vi "Event Handler.vi"(0 "uService Template in":refnum<class "Error Manager.lvclass">, 5 "Event type":T1=enum."Message", 7 "Item Name":string, 9 "Data":variant, 11 "error in (no error)":errorcluster) -> (4 "uService Template out":refnum<class "Error Manager.lvclass">, 15 "error out":errorcluster)   [LabVIEW 2020, in "TALOS.lvlib" / "Error Manager.lvlib" / "Error Manager.lvclass"]
doc: "This VI is the event handler of the uService: every time an event is triggered to the uService, this VI is called.\nNote: here you can access the Actor/Class data, but it will be the one coming out from Init. You cannot modify the values.\nThree different events are supported:\nI) Button Pressed: get called on a GUI button pressed. Item Name is the name (label) of the button, Data is empty.\nII) Shared Variable Updated: get called when a SV you subscribed to is updated. Item Name is the name of the SV, and Data is the value (note: you need to convert it to the proper type).\nIII) Message: get called every time a user event is generated using Send Message to Event Handler. The values of Item Name and Data are the one given to the Send Message to Event Handler.\nIV) Ready to launch?: this frame get called every time a new Run is initiated. Each uService is responsible of performing a self check before giving back the green light for the Run to start."
uses:
  Error Manager.lvclass
  C:/Users/marco/Documents/GitHub_Lab/TALOS/talos/Father of all uServices/Father of all uServices/Father of all uServices.lvclass
  Father of all uServices/Father of all uServices/Event Handler Items.ctl
  Ancestor/Ancestor/Ancestor.lvclass/Ancestor.ctl
  Error Manager Consumer Case Selector.ctl
  Father of all uServices/Father of all uServices Messages/Consumer Msg/Consumer Msg.lvclass/Consumer Msg.ctl
  Error Info.ctl
  Father of all uServices/Father of all uServices/Father of all uServices.lvclass/Father of all uServices.ctl
  FGV/Error Memory/Get Error Description.vi
  Support VIs/Get PC name.vi
  Ancestor/Ancestor/Read ID.vi
  Support VIs/Get Class Name.vi
  <vilib>/Utility/error.llb/Clear Errors.vi
  Father of all uServices/Father of all uServices Messages/Consumer Msg/Send Consumer.vi
  FGV/Error Memory/Error Memory Core.vi
  <vilib>/AdvancedString/Delimited String to 1D String Array.vi
  Support VIs/Circus Root Path.vi
  FGV/Error Memory/Error Crt Lvl checker.vi
  FGV/Error Memory/Error Memory Core.vi/40c8088d-b597-4017-91af-faa98e00292e.vi
  FGV/Error Memory/Error Memory Core.vi/d4a3ab98-063c-4e44-b43d-fbdcfe6c2be2.vi
  Father of all uServices/Father of all uServices/Father of all uServices.lvclass
  C:/Users/marco/Documents/GitHub_Lab/TALOS/builds/Actor Framework PPL/Actor Framework.lvlibp/1abvi3w/vi.lib/ActorFramework/Actor/Actor.lvclass
  Support VIs/Global Memory.vi
  <vilib>/Utility/LVClass/Get LV Class Name.vi
  Support VIs/Is in Packed Library.vi
  Support VIs/TALOS Root path.vi
  Support VIs/Read CSV worksheet.vi
  Support VIs/Global Constants.vi
  <vilib>/Utility/error.llb/General Error Handler.vi
  Support VIs/Error Log.vi
  builds/Actor Framework PPL/Actor Framework.lvlibp/1abvi3w/vi.lib/ActorFramework/Actor/Read Self Enqueuer.vi
  <userlib>/_OpenG.lib/lvdata/lvdata.llb/Get Strings from Enum__ogtk.vi
  builds/Actor Framework PPL/Actor Framework.lvlibp/1abvi3w/vi.lib/ActorFramework/Message Enqueuer/Enqueue.vi
  Ancestor/Ancestor/Ancestor.lvclass
  <vilib>/Comparison/Equal/Equal Functor/Equal Functor.lvclass
  Father of all uServices/Father of all uServices Messages/Consumer Msg/Consumer Msg.lvclass
  Error Manager.lvclass/Error Manager.ctl
  TALOS.lvlib
  FGV/Error Memory/Error Memory.lvlib
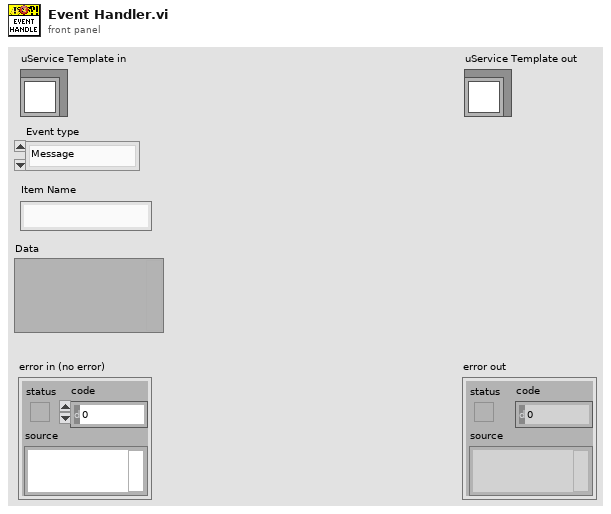
[diagram p1: front panel]
types:
  T1 = typedef "TALOS.lvlib/Father of all uServices.lvlib/Father of all uServices.lvclass/Event Handler Items.ctl" = enum16{"Button Pressed", "Message", "Ready to launch?", "Safe Mode", "Start RUN", "Stop RUN"}
  T2 = typedef "TALOS.lvlib/Error Manager.lvlib/Error Manager.lvclass/Error Manager Consumer Case Selector.ctl" = enum16{"Init", "Digest Error", "Dismiss Error", "Dismiss All", "Show Error Details", "Filter out Errors", "Clear Filters"}
  T3 = typedef "TALOS.lvlib/Error Manager.lvlib/Error Manager.lvclass/Error Info.ctl" = cluster{"error out":errorcluster, "Time Stamp":timestamp, "Machine Name":string, "GUID":string}
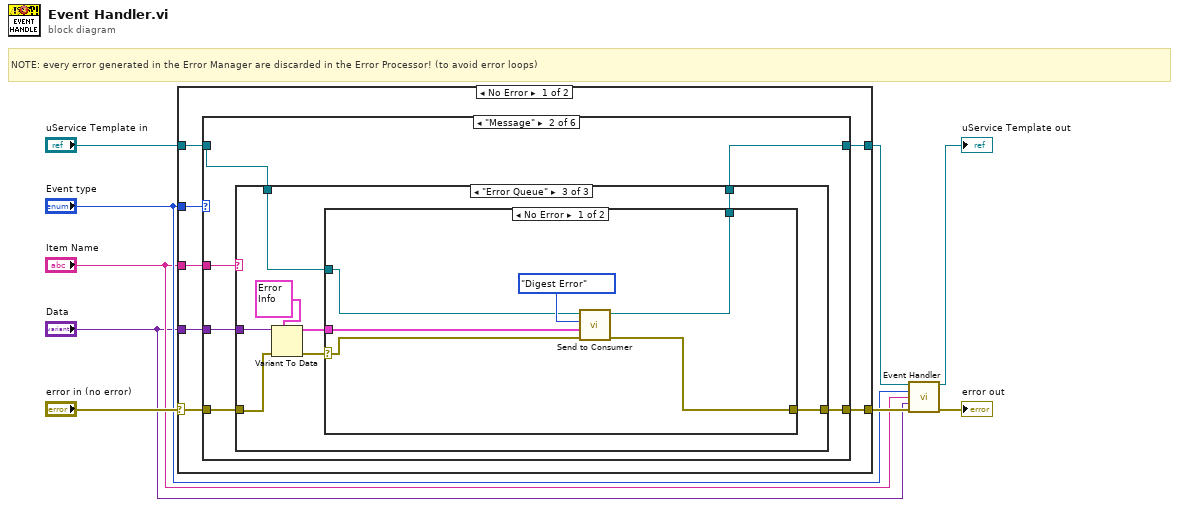
[diagram p0: block diagram]
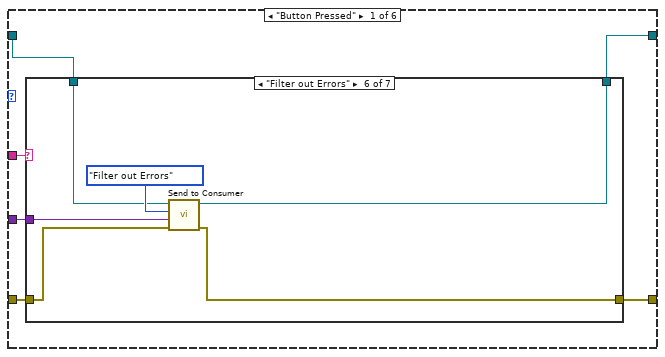
[diagram p2: hidden frame]
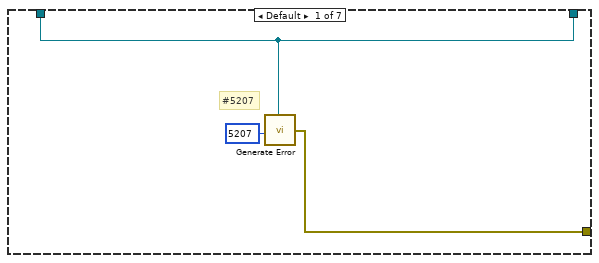
[diagram p3: hidden frame]
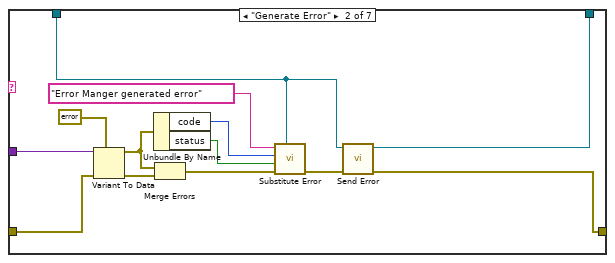
[diagram p4: hidden frame]
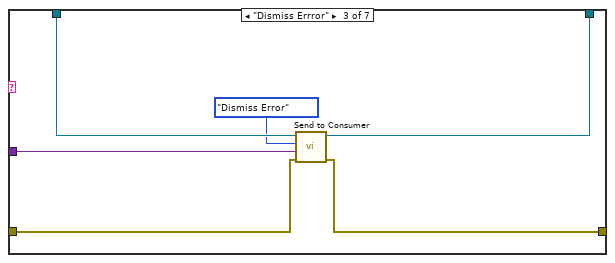
[diagram p5: hidden frame]
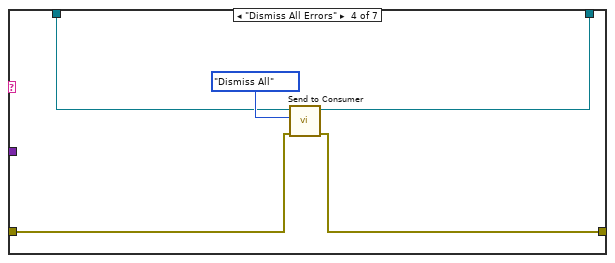
[diagram p6: hidden frame]
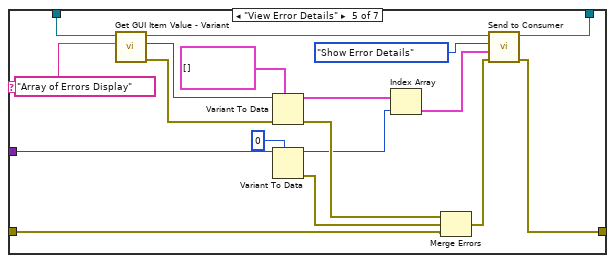
[diagram p7: hidden frame]
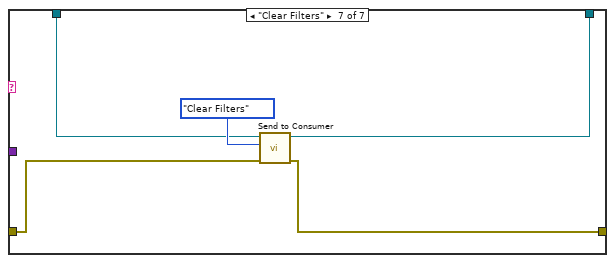
[diagram p8: hidden frame]
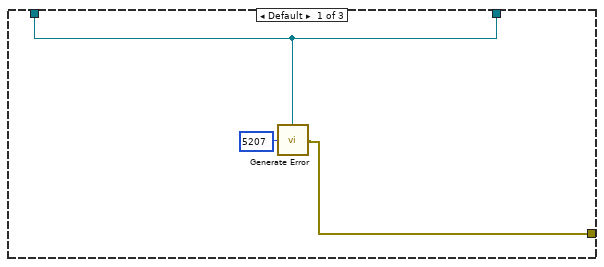
[diagram p9: hidden frame]
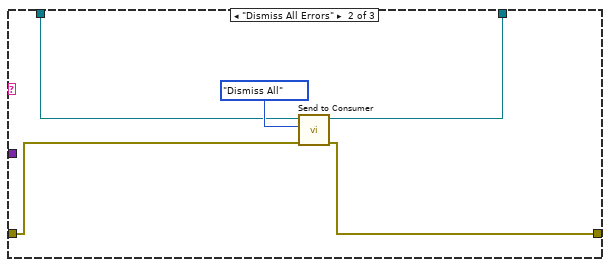
[diagram p10: hidden frame]
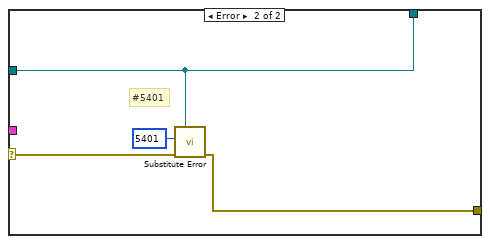
[diagram p11: hidden frame]
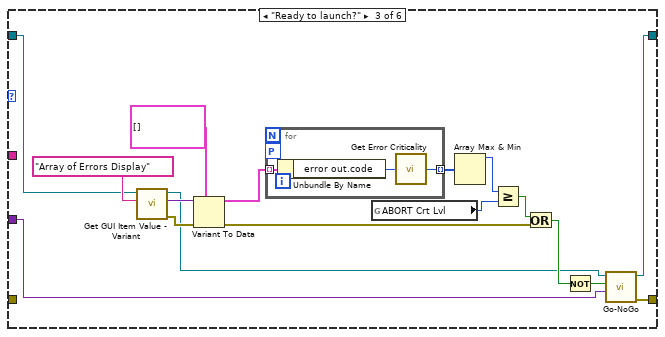
[diagram p12: hidden frame]
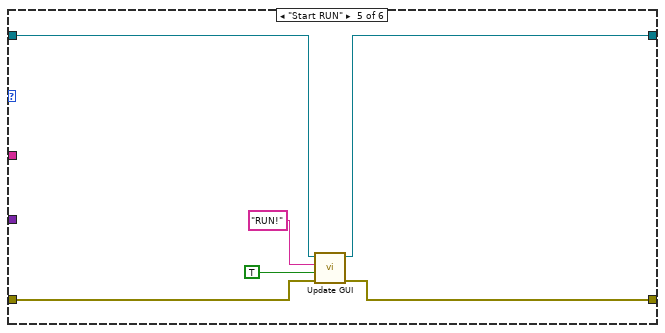
[diagram p14: hidden frame]
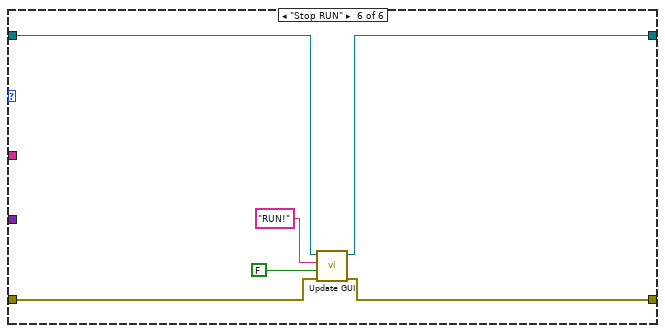
[diagram p15: hidden frame]
diagram:
  # "NOTE: every error generated in the Error Manager are discarded in the Error Processor! (to avoid error loops)"
  n1 = case shown="No Error" "error in (no error)" {
    selector: "error in (no error)" -> [w14 w146]
    tunnel: [w15 w146] -> w7
    tunnel: [w10 w145] -> w4
    tunnel: "uService Template in" -> [w13 w145]
    tunnel: "Event type" -> [w16 _]
    tunnel: "Item Name" -> [w12 _]
    tunnel: "Data" -> [w11 _]
    frame No Error {
      n2 = case shown="\"Message\"" w16 {
        tunnel: [w22 w80 w124 w132 w138 w144] -> w15
        tunnel: w14 -> [w19 w84 _ w132 w137 w143]
        tunnel: w12 -> [w20 w83 _ _ _ _]
        tunnel: w13 -> [w21 w81 w123 w131 w134 w140]
        tunnel: w11 -> [w18 w82 w113 _ _ _]
        tunnel: [w17 w79 w111 w131 w133 w139] -> w10
        frame "Button Pressed" {
          n3 = case shown="\"Filter out Errors\"" w20 {
            tunnel: w19 -> [_ w36 w42 w47 w52 w71 w76]
            tunnel: [w24 w37 w41 w46 w59 w70 w75] -> w22
            tunnel: w21 -> [w23 w33 w44 w48 w63 w72 w77]
            tunnel: w18 -> [_ w34 w40 _ w57 w69 _]
            tunnel: [w23 w26 w39 w45 w50 w68 w74] -> w17
            frame Default {
              # "#5207"
              n4 = call "Generate Error.vi"("Class"=w23, "Error Code"=5207) -> ("error out"=w24:errorcluster)  [unwired: 5 in]
            }
            frame "Generate Error" {
              n5 = Variant To Data(error in=w36, type=errorcluster {"status"=FALSE, "code"=0, "source"=""} ("error IO"), Variant=w34) -> (data=w30:errorcluster, error out=w38:errorcluster)
              n6 = Unbundle By Name(w30) -> ("code"=w29:i32, "status"=w28:bool)
              n7 = Merge Errors(w30, w38) -> (w32:errorcluster)
              n8 = call "Substitute Error.vi"("LabVIEW Object"=w33, "error in (no error)"=w32, "Error/Warning"=w28, "Error Code"=w29, "Optional String"="Error Manger generated error") -> ("error out"=w31:errorcluster)  [unwired: 6 in]
              n9 = call-dynamic "Send Error.vi"("error in (no error)"=w31, "Father of all uServices in"=w33) -> ("error out"=w37:errorcluster, "Father of all uServices out"=w26:refnum<class "Error Manager.lvclass">)  [unwired: 8 in]
            }
            frame "Dismiss Errror" {
              n10 = call "Send to Consumer.vi"("error in (no error)"=w42, "Data"=w40, "Case ID"=Error_Manager_Consumer_Case_Selector."Dismiss Error" ("ErrMgr Case Selector"), "uService Template in"=w44) -> ("error out"=w41:errorcluster, "uService Template out"=w39:refnum<class "Error Manager.lvclass">)  [unwired: 6 in]
            }
            frame "Dismiss All Errors" {
              n11 = call "Send to Consumer.vi"("error in (no error)"=w47, "Case ID"=Error_Manager_Consumer_Case_Selector."Dismiss All" ("ErrMgr Case Selector"), "uService Template in"=w48) -> ("error out"=w46:errorcluster, "uService Template out"=w45:refnum<class "Error Manager.lvclass">)  [unwired: 7 in]
            }
            frame "View Error Details" {
              n12 = call "Get GUI Item Value - Variant.vi"("FP Item Name"="Array of Errors Display", "uService Template in"=w63) -> ("error out"=w62:errorcluster, "Value"=w61:variant, "uService Template out"=w58:refnum<class "Error Manager.lvclass">)  [unwired: 7 in]
              n13 = Variant To Data(error in=w62, type=T3[] [] ("error constant"), Variant=w61) -> (data=w65:T3[], error out=w67:errorcluster)
              n14 = Variant To Data(type=0 ("Select Error"), Variant=w57) -> (data=w54:i32, error out=w53:errorcluster)  [unwired: 1 in]
              n15 = Index Array(array=w65, index=w54) -> (element=w55:T3)
              n16 = Merge Errors(w67, w53, w52) -> (w51:errorcluster)
              n17 = call "Send to Consumer.vi"("error in (no error)"=w51, "Data"=w55, "Case ID"=Error_Manager_Consumer_Case_Selector."Show Error Details" ("ErrMgr Case Selector"), "uService Template in"=w58) -> ("error out"=w59:errorcluster, "uService Template out"=w50:refnum<class "Error Manager.lvclass">)  [unwired: 6 in]
            }
            frame "Filter out Errors" {
              n18 = call "Send to Consumer.vi"("error in (no error)"=w71, "Data"=w69, "Case ID"=Error_Manager_Consumer_Case_Selector."Filter out Errors" ("ErrMgr Case Selector"), "uService Template in"=w72) -> ("error out"=w70:errorcluster, "uService Template out"=w68:refnum<class "Error Manager.lvclass">)  [unwired: 6 in]
            }
            frame "Clear Filters" {
              n19 = call "Send to Consumer.vi"("error in (no error)"=w76, "Case ID"=Error_Manager_Consumer_Case_Selector."Clear Filters" ("ErrMgr Case Selector"), "uService Template in"=w77) -> ("error out"=w75:errorcluster, "uService Template out"=w74:refnum<class "Error Manager.lvclass">)  [unwired: 7 in]
            }
          }
        }
        frame "Message" {
          n20 = case shown="\"Error Queue\"" w83 {
            tunnel: w84 -> [_ w90 w95]
            tunnel: w82 -> [_ _ w94]
            tunnel: w81 -> [w85 w91 w96]
            tunnel: [w87 w89 w97] -> w80
            tunnel: [w85 w88 w93] -> w79
            frame Default {
              n21 = call "Generate Error.vi"("Class"=w85, "Error Code"=5207) -> ("error out"=w87:errorcluster)  [unwired: 5 in]
            }
            frame "Dismiss All Errors" {
              n22 = call "Send to Consumer.vi"("error in (no error)"=w90, "Case ID"=Error_Manager_Consumer_Case_Selector."Dismiss All" ("ErrMgr Case Selector"), "uService Template in"=w91) -> ("error out"=w89:errorcluster, "uService Template out"=w88:refnum<class "Error Manager.lvclass">)  [unwired: 7 in]
            }
            frame "Error Queue" {
              n23 = Variant To Data(error in=w95, type=T3 {"error out"={"status"=FALSE, "code"=0, "source"=""}, "Time Stamp"=timestamp(0 s since 1904-01-01), "Machine Name"="", "GUID"=""} ("Error Info"), Variant=w94) -> (data=w99:T3, error out=w100:errorcluster)
              n24 = case shown="No Error" w100 {
                selector: w100 -> [w105 w110]
                tunnel: w96 -> [w102 w107]
                tunnel: [w106 w109] -> w97
                tunnel: w99 -> [w104 _]
                tunnel: [w101 w107] -> w93
                frame No Error {
                  n25 = call "Send to Consumer.vi"("error in (no error)"=w105, "Data"=w104, "Case ID"=Error_Manager_Consumer_Case_Selector."Digest Error" ("ErrMgr Case Selector"), "uService Template in"=w102) -> ("error out"=w106:errorcluster, "uService Template out"=w101:refnum<class "Error Manager.lvclass">)  [unwired: 6 in]
                }
                frame Error {
                  # "#5401"
                  n26 = call "Substitute Error.vi"("LabVIEW Object"=w107, "error in (no error)"=w110, "Error Code"=5401) -> ("error out"=w109:errorcluster)  [unwired: 8 in]
                }
              }
            }
          }
        }
        frame "Ready to launch?" {
          n27 = call "Get GUI Item Value - Variant.vi"("FP Item Name"="Array of Errors Display", "uService Template in"=w123) -> ("error out"=w122:errorcluster, "Value"=w126:variant, "uService Template out"=w112:refnum<class "Error Manager.lvclass">)  [unwired: 7 in]
          n28 = Variant To Data(error in=w122, type=T3[] [] ("error constant"), Variant=w126) -> (data=w121:T3[], error out=w117:errorcluster)
          n29 = for {
            tunnel: w121 -> [w130] mode=indexing
            workers-P: _ -> [_]
            tunnel: [w128] -> w120 mode=indexing
            n30 = Unbundle By Name(w130) -> ("error out.code"=w129:i32)
            n31 = call "Get Error Criticality.vi"("Error Code in"=w129) -> ("Error Criticality"=w128:u8)  [unwired: 4 in]
          }
          n32 = global read "Global Constants.vi" "ABORT Crt Lvl"() -> (w114:u8)
          n33 = Array Max & Min(array=w120) -> (max value=w119:u8)  [unwired: 3 out]
          n34 = Greater Or Equal?(x=w119, y=w114) -> (x >= y?=w118:bool)
          n35 = Or(x=w118, y=w117) -> (x .or. y?=w115:bool)
          n36 = Not(x=w115) -> (.not. x?=w116:bool)
          n37 = call-dynamic "Go-NoGo.vi"("Go-NoGo Data"=w113, "Go?"=w116, "Father of all uServices in"=w112) -> ("error out"=w124:errorcluster, "Father of all uServices out"=w111:refnum<class "Error Manager.lvclass">)  [unwired: 7 in]
        }
        frame "Safe Mode" {
        }
        frame "Start RUN" {
          n38 = call "Update GUI.vi"("error in (no error)"=w137, "Data"=TRUE ("Go?"), "GUI Item Name"="RUN!", "uService Template in"=w134) -> ("error out"=w138:errorcluster, "uService Template out"=w133:refnum<class "Error Manager.lvclass">)  [unwired: 6 in]
        }
        frame "Stop RUN" {
          n39 = call "Update GUI.vi"("error in (no error)"=w143, "Data"=FALSE ("Go?"), "GUI Item Name"="RUN!", "uService Template in"=w140) -> ("error out"=w144:errorcluster, "uService Template out"=w139:refnum<class "Error Manager.lvclass">)  [unwired: 6 in]
        }
      }
    }
    frame Error {
    }
  }
  n40 = call-parent "Event Handler.vi"("uService Template in"=w4, "Event type"="Event type", "Item Name"="Item Name", "Data"="Data", "error in (no error)"=w7) -> ("uService Template out"=→"uService Template out":refnum<class "Error Manager.lvclass">, "error out"=→"error out":errorcluster)  [unwired: 9 in]
